vi "Write Variable.vi"   [LabVIEW 2019, in "LV-Data.PGSQL.lvclass"]
uses:
  LV-Data.PGSQL.lvclass
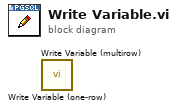
[diagram p0: block diagram]
diagram:
  n1 = call "Write Variable (one-row).vi"() -> ()  [unwired: 8 in, 4 out]
  n2 = call "Write Variable (multirow).vi"() -> ()  [unwired: 8 in, 4 out]
